vi "距离测量 - DS.vi"(7 "CSM Name":string="DS1") -> ()   [LabVIEW 2026, in "UI-距离测量.lvlib"]
uses:
  Supports/Sample Settings.ctl
  Data ColndSave/Supports/Time and Data.ctl
  TCP/Supports/UDP Settings.ctl
  <userlib>/_NEVSTOP/Communicable State Machine(CSM)/_Polymophic/CSM - Filter Duplicated Lines.vi
  aad2107a-5a5f-4fdf-8db0-9c36fd42b832.vi
  0bbdcba1-9d5b-49e3-b023-81a6ed1a833f.vi
  d3182339-f607-4847-9390-ad77bbb9bef6.vi
  a3283b4f-3d7d-475f-8286-b95f18be6a9d.vi
  b77c2947-8455-45d0-8563-f45fdc66c63a.vi
  c6692627-02fb-4556-9c5d-59e6097d0856.vi
  8c0fc226-3871-4866-9b38-f175316b3ef9.vi
  8417ea6c-3bd9-4cd5-8933-b29b0935beb3.vi
  <userlib>/_NEVSTOP/Communicable State Machine(CSM)/_Polymophic/CSM - Replace Marks in Messages.vi
  9e8a82e7-73dc-49c7-a8e1-da740b95007e.vi
  45363da5-0a68-41f0-863f-59b1647d93dc.vi
  684e6125-f2cc-419b-bab0-170e1ce567bd.vi
  5163a33a-69e0-492d-a74e-a390bdb1a610.vi
  3f58c0c9-4519-4815-81b6-823063e0ea10.vi
  ed6ed594-6bdd-4916-8b11-5c87dc2a661e.vi
  f090f7de-5b96-425f-bcc2-868efcdef004.vi
  7a757d38-3930-42d9-9f77-20f8f863129d.vi
  d1e74b47-9369-4dfd-ba75-b02d04b7ee9f.vi
  ba09a988-f7d6-44f3-a6d8-47fd2b4ee3b5.vi
  4c4982bb-7a2e-4137-8dbb-56eff7d2cb39.vi
  d32f4df3-bc1c-40d9-8b4f-fe0ac986a064.vi
  <userlib>/_NEVSTOP/Communicable State Machine(CSM)/AdvanceAPI/CSM - Compact Multiple States.vi
  <userlib>/_NEVSTOP/Communicable State Machine(CSM)/AdvanceAPI/CSM - Break Down Multiple States String.vi
  <userlib>/_NEVSTOP/Communicable State Machine(CSM)/_Shared/Remove Comments from Single-line.vi
  <userlib>/_NEVSTOP/Communicable State Machine(CSM)/_Shared/Split Single-line Message.vi
  <userlib>/_NEVSTOP/Communicable State Machine(CSM)/_Shared/Trim Single-line Text.vi
  <userlib>/_NEVSTOP/Communicable State Machine(CSM)/AdvanceAPI/CSM - Revert Arguments-Safe String.vi
  <userlib>/_NEVSTOP/Communicable State Machine(CSM)/AdvanceAPI/CSM - Make String Arguments Safe.vi
  c6692627-02fb-4556-9c5d-59e6097d0856.vi/99de0c97-112a-4c86-9094-c187659127e1.vi
  <userlib>/_NEVSTOP/Communicable State Machine(CSM)/Utility/Build Error Cluster.vi
  8417ea6c-3bd9-4cd5-8933-b29b0935beb3.vi/99de0c97-112a-4c86-9094-c187659127e1.vi
  <userlib>/_NEVSTOP/Communicable State Machine(CSM)/AdvanceAPI/CSM - Keywords.vi
  <userlib>/_NEVSTOP/Communicable State Machine(CSM)/addons/API-String-Arugments-Support/_Support/Data To API String Arguments.vi
  <userlib>/_NEVSTOP/Communicable State Machine(CSM)/addons/INI-Static-Variable-Support/_Support/instances/_CSM - Read File Logger Configuration - v1.0.vi
  <vilib>/Utility/Data Type/Get Type Information.vi
  <userlib>/_NEVSTOP/Communicable State Machine(CSM)/addons/API-String-Arugments-Support/_Support/Data To SingleElementsArray_csm.vi
  <userlib>/_NEVSTOP/Communicable State Machine(CSM)/addons/INI-Static-Variable-Support/_Support/Parse Used Session and Name.vi
  <userlib>/_NEVSTOP/Communicable State Machine(CSM)/addons/INI-Static-Variable-Support/_Support/INI-FGV(lvlibp).vi
  <userlib>/_NEVSTOP/Communicable State Machine(CSM)/addons/INI-Static-Variable-Support/_Support/Populate String with INI Variable.vi
  <userlib>/_NEVSTOP/Communicable State Machine(CSM)/addons/API-String-Arugments-Support/_Support/Convert API String Arguments to Data(variant).vi
  <userlib>/_NEVSTOP/Communicable State Machine(CSM)/addons/API-String-Arugments-Support/_Support/SingleElementsArray To Data_csm.vi
  <userlib>/_NEVSTOP/Communicable State Machine(CSM)/addons/MassData-Parameter/_support/FGV-MassData(lvlibp).vi
  <vilib>/Instr/_visa.llb/VISA Configure Serial Port (Instr).vi
  <userlib>/_NEVSTOP/Communicable State Machine(CSM)/Communicable State Machine.lvlib
  Acquisition/Acquisition.lvlib
  <userlib>/_NEVSTOP/Communicable State Machine(CSM)/addons/MassData-Parameter/CSM MassData Parameter Support.lvlib
  <userlib>/_NEVSTOP/Communicable State Machine(CSM)/addons/INI-Static-Variable-Support/INI-Static-Variable-Support.lvlib
  <userlib>/_NEVSTOP/Communicable State Machine(CSM)/addons/Watchdog/CSM Watchdog.lvlib
  <userlib>/_NEVSTOP/Communicable State Machine(CSM)/addons/Logger/CSM File Logger.lvlib
  Logging/Logging.lvlib
  Data ColndSave/Data Collection and Save.lvlib
  TCP/UDP.lvlib
panel:
  in  "停止":bool
  in  "温度显示":enum32{"距离测量", "Status"}(tab)
  in  "地址":string
  in  "UDP":bool
  in  "光功率模式":bool
  in  "光功率设置":u32
  in  "光开关":bool
  in  "距离采集开关":bool
  in  "USB Port":refnum<visa-resource-name>="COM3"
  in  "Interval(s)":dbl=0.5
  out "距离":waveform(dbl)(graph)
  in  "子程序？":bool
  out "Error Occurred":errorcluster caption="温度采集-错误输出"
  out "State History":string
  # "(5-1000)"
  # "mm"
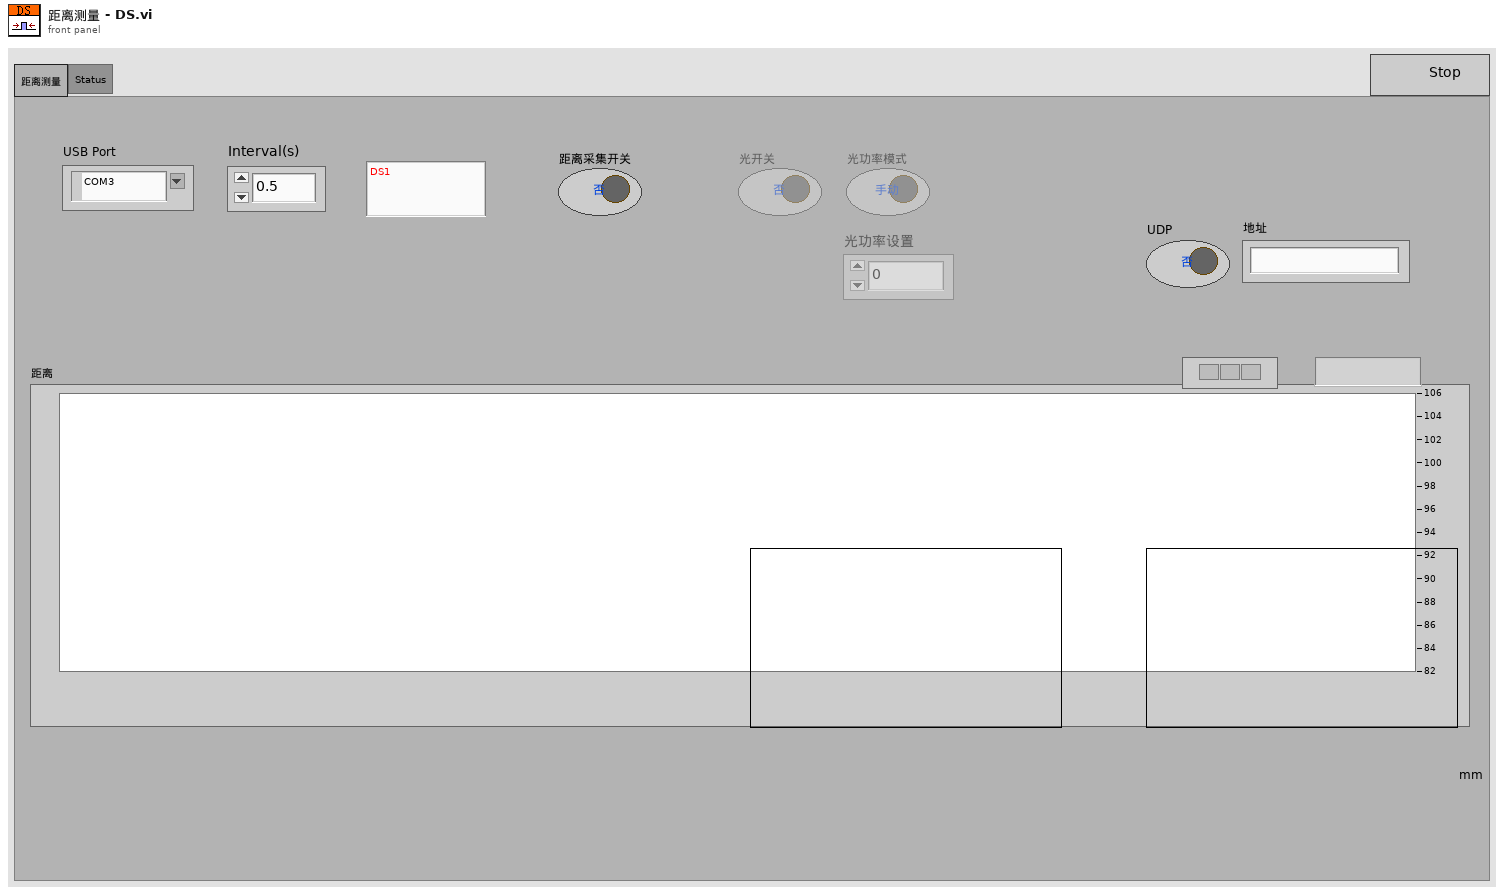
[diagram p1: front panel]
types:
  T1 = cluster{"Enable":bool, "Limit":cluster{"FileSize":i64, "FileNum":i32}, "Timestamp.Format":string, "AutoExit":bool}
  T2 = enum32{"Invalid", "Standard", "Closed", "Hidden", "Minimized", "Maximized"}
  T3 = enum32{"invalid app kind", "Development System", "Run Time System", "Student Edition", "Embedded LabVIEW", "Evaluation", "Custom"}
  T4 = cluster{"波特率":u32, "数据位":u16, "校验":enum16{"None", "Odd", "Even", "Mark", "Space"}, "停止位":u16, "流控制":u16}
  T5 = typedef "UI-距离测量.lvlib/读写指令类型.ctl" = enum16{"03读保持寄存器", "04读输入寄存器", "06写单个寄存器"}
  T6 = typedef "UI-距离测量.lvlib/UDP.lvlib/UDP Settings.ctl" = cluster{"连接ID":refnum<k16>, "网络地址(字符串)":string, "地址":u32, "本端口":u16, "对向":u16, "Read Interval":dbl, "Write Interval":dbl}
  T7 = typedef "Communicable State Machine.lvlib/_CSM_Response Source Message.ctl" = cluster{"‘State":string, "’Arguments":string, "’Error":errorcluster}
  T8 = cluster{"Current VI Reference":refnum<vi>, "Close Panel on Exit?":bool}
  T9 = typedef "UI-距离测量.lvlib/Sample Settings.ctl" = cluster{"USB Port":refnum<visa-resource-name>, "Interval(s)":dbl}
  T10 = typedef "Data Collection and Save.lvlib/Time and Data.ctl" = cluster{"采集时间":timestamp, "Data":dbl[]}
  T11 = cluster{"Core":cluster{"Current VI Reference":refnum<vi>, "Close Panel on Exit?":bool}, "Sample Settings":T9, "Time and Data":T10, "子程序？":bool}
  T12 = enum8{"Enabled", "Disabled", "Disabled and Grayed Out"}
  T13 = typedef "全局变量数据.ctl" = cluster{"温度采集":dbl[], "温度控制":dbl[], "压力测量":dbl[], "Zolix":dbl[], "步进电机":dbl[], "湿度测量":dbl[], "距离测量":dbl[]}
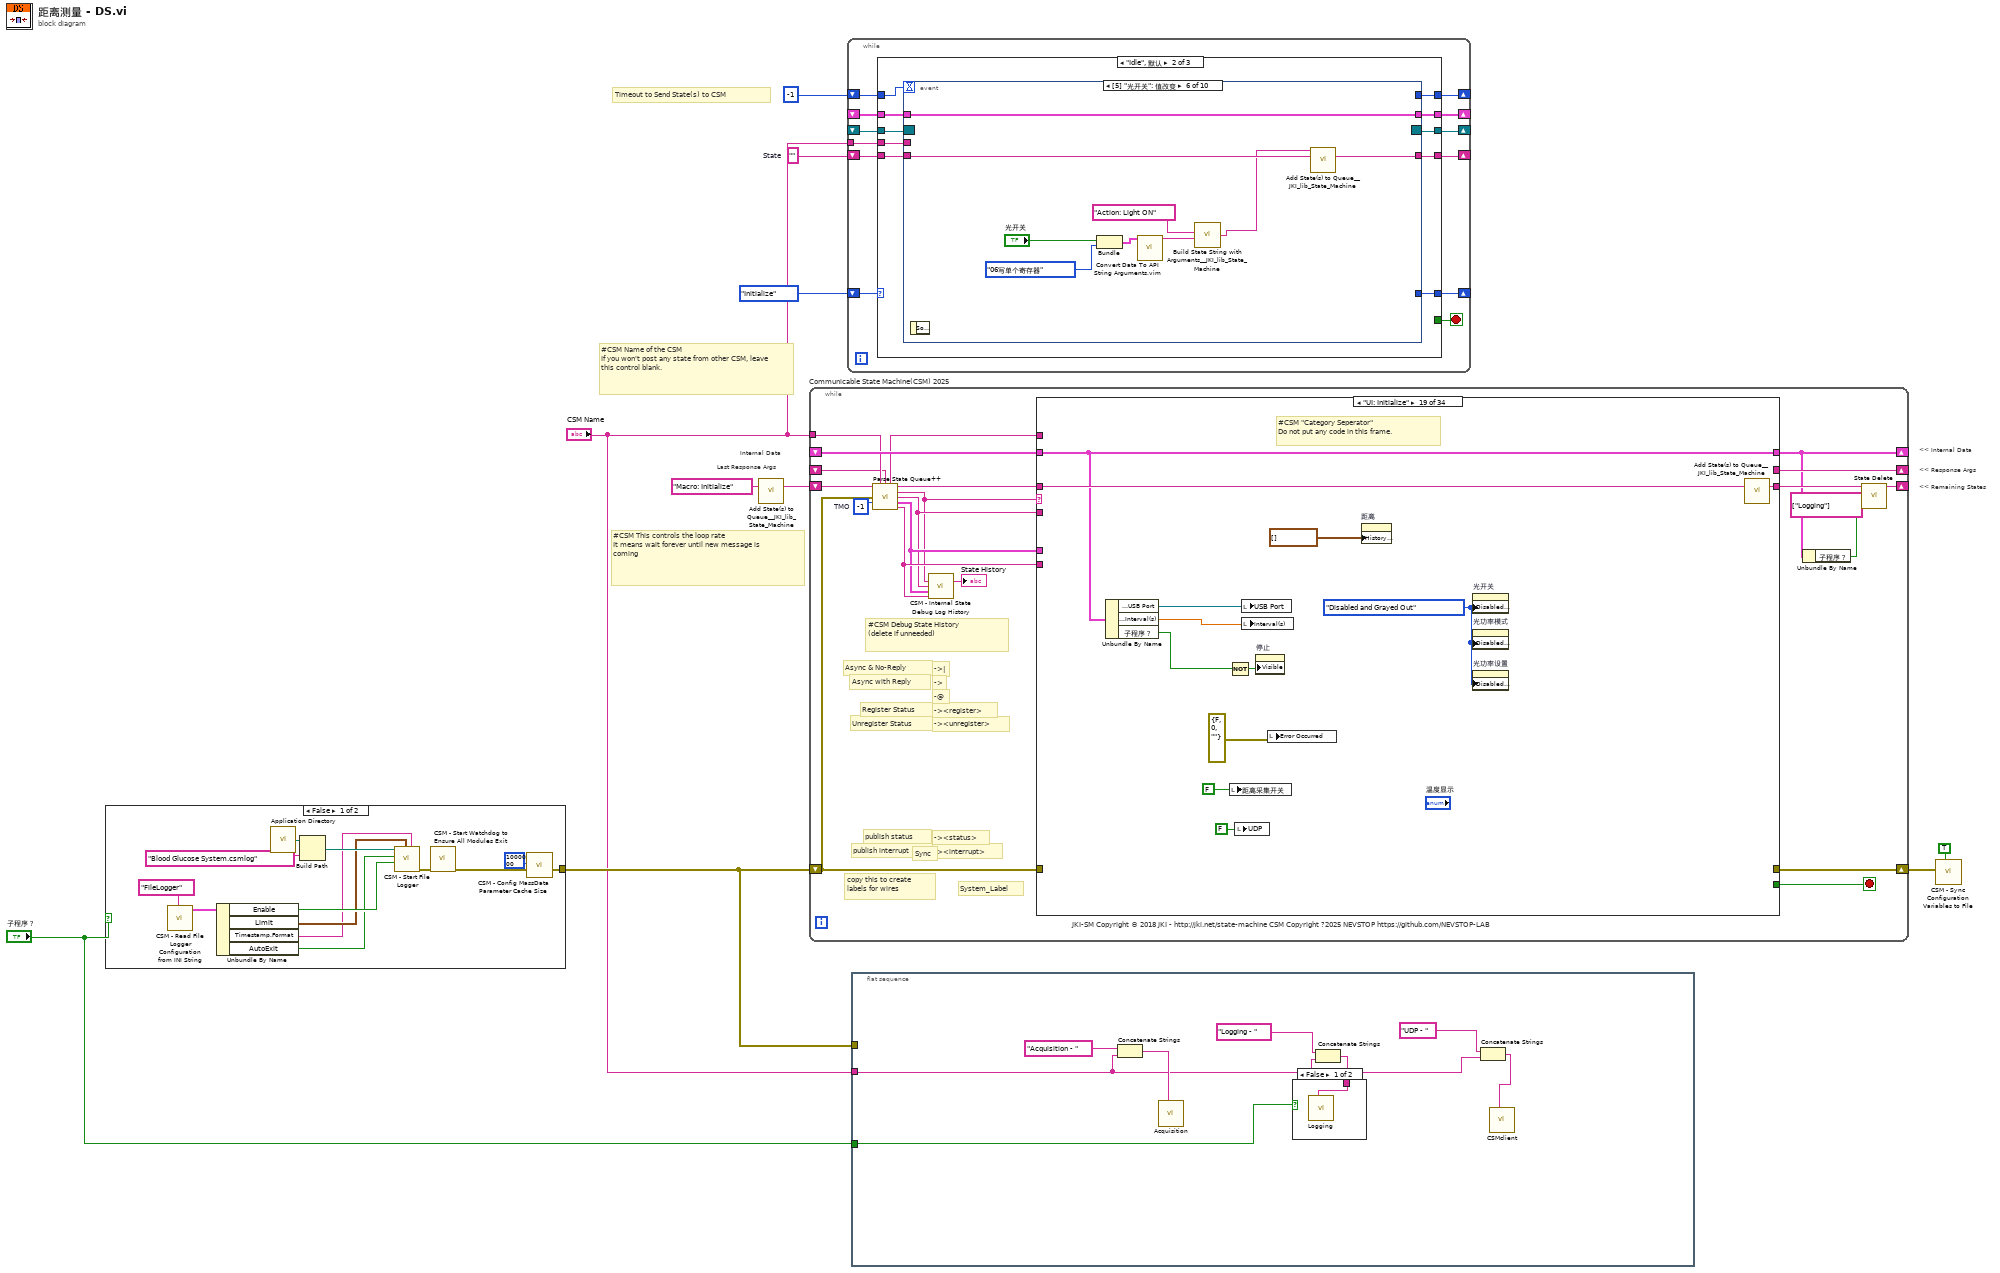
[diagram p0: block diagram]
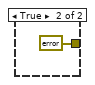
[diagram p2: hidden frame]
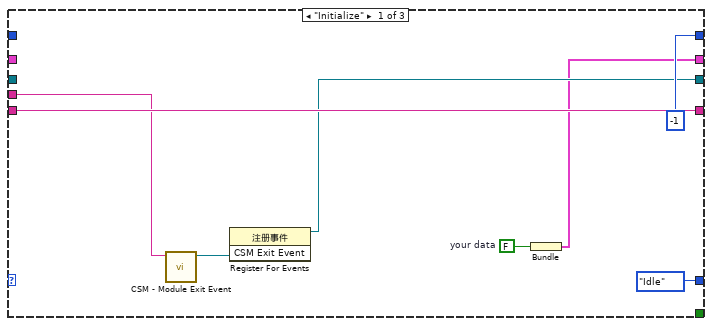
[diagram p4: hidden frame]
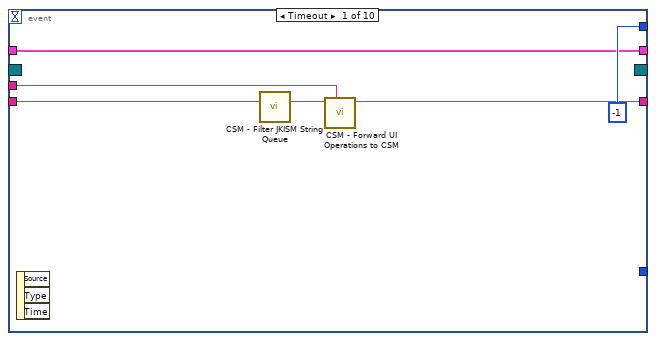
[diagram p5: hidden frame]
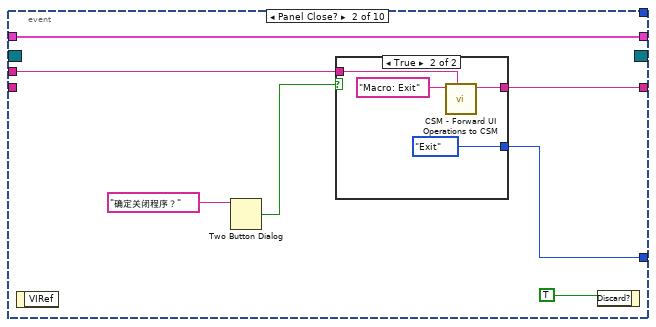
[diagram p6: hidden frame]
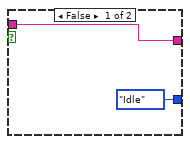
[diagram p7: hidden frame]
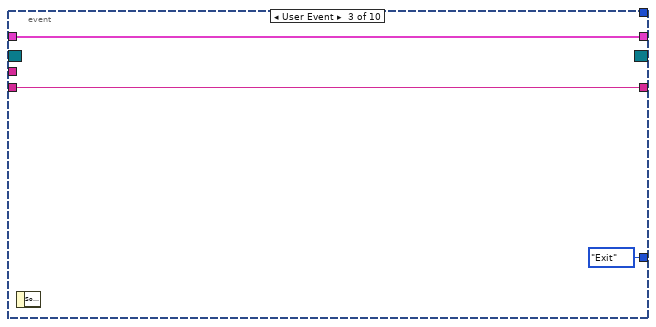
[diagram p8: hidden frame]
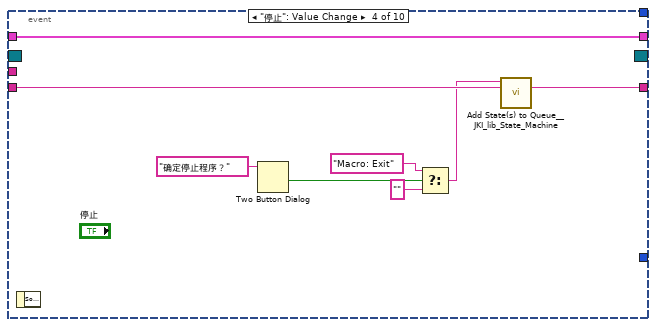
[diagram p9: hidden frame]
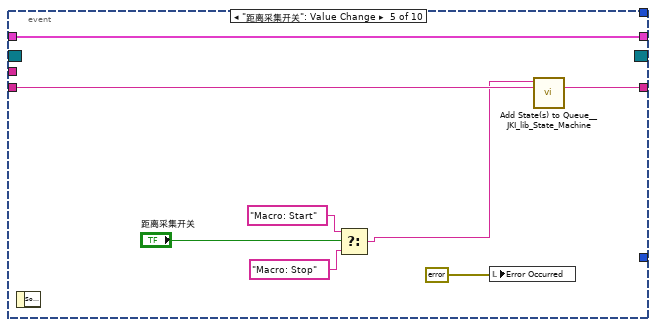
[diagram p10: hidden frame]
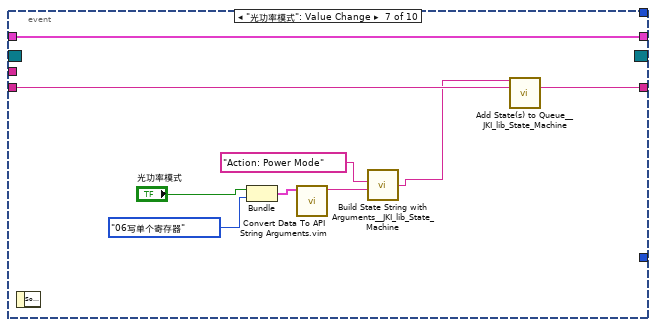
[diagram p11: hidden frame]
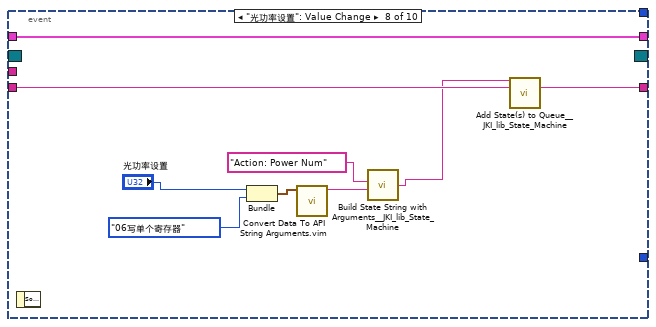
[diagram p12: hidden frame]
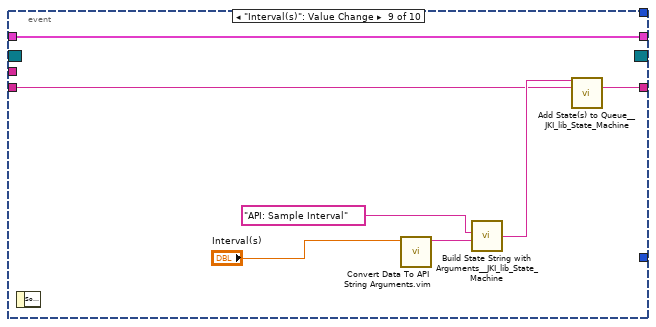
[diagram p13: hidden frame]
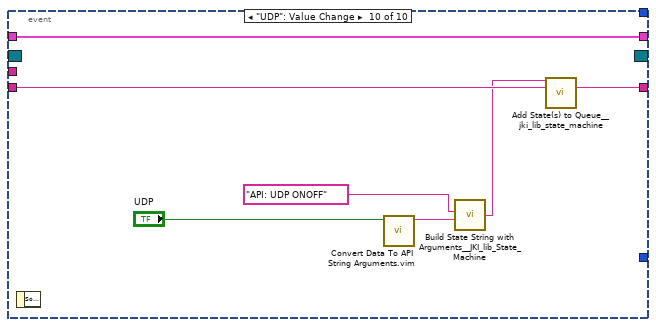
[diagram p14: hidden frame]
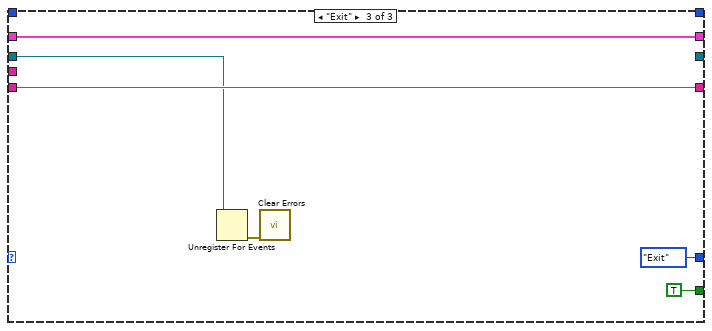
[diagram p15: hidden frame]
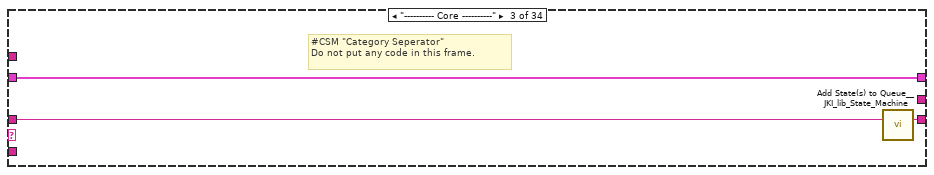
[diagram p18: hidden frame]
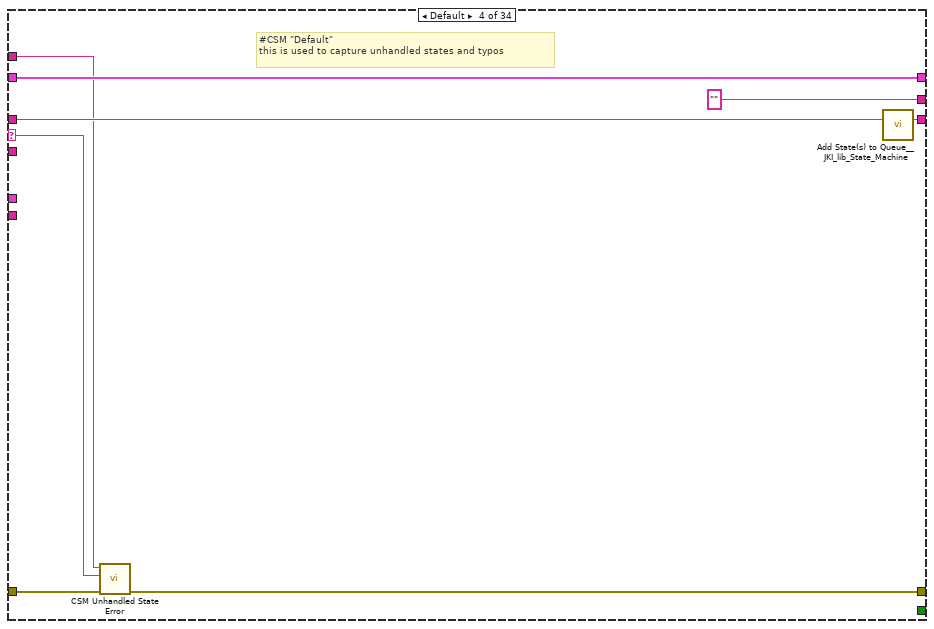
[diagram p19: hidden frame]
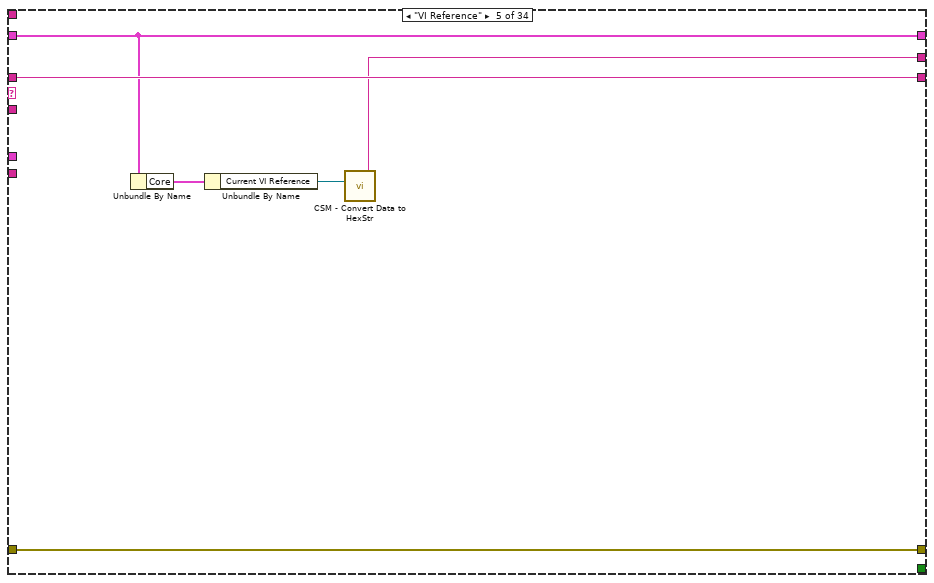
[diagram p20: hidden frame]
diagram:
  w9 = ""  # State
  # "Timeout to Send State(s) to CSM"
  # "Last Response Args"
  # "Internal Data"
  # "#CSM Name of the CSM\nIf you won't post any state from other CSM, leave this control blank."
  # "#CSM This controls the loop rate\nIt means wait forever until new message is coming"
  # "<< Internal Data"
  # "<< Response Args"
  # "<< Remaining States"
  n1 = case shown="False" "子程序？" {
    tunnel: [w11 errorcluster {"status"=FALSE, "code"=0, "source"=""} ("Error out")] -> w5
    frame False {
      n2 = call-poly <userlib>:"CSM - Read File Logger Configuration from INI String.vi"("Section Name(\"FileLogger\")"="FileLogger" ("Section Name(\"\" as Default)")) -> ("FileLogger Configuration-v1"=w18:T1)  [unwired: 7 in, 1 out]
      n3 = Unbundle By Name(w18) -> ("Enable"=w17:bool, "Limit"=w16:cluster{"FileSize":i64, "FileNum":i32}, "Timestamp.Format"=w14:string, "AutoExit"=w15:bool)
      n4 = call <vilib>:"Application Directory.vi"() -> ("Application Directory"=w23:path)
      n5 = Build Path(base path=w23, name or relative path="Blood Glucose System.csmlog") -> (appended path=w21:path)
      n6 = call <userlib>:"CSM - Start File Logger.vi"("Timestamp Format"=w14, "Log Limit"=w16, "Watchdog? (T)"=w17, "Exit When All Module Exist? (F)"=w15, "Log File Path"=w21) -> ("error out"=w20:errorcluster)  [unwired: 4 in, 2 out]
      n7 = call <userlib>:"CSM - Start Watchdog to Ensure All Modules Exit.vi"("error in (no error)"=w20) -> ("error out"=w12:errorcluster)  [unwired: 10 in]
      n8 = call <userlib>:"CSM - Config MassData Parameter Cache Size.vi"("Error in"=w12, "Size (50M)"=1000000 ("size(1M)")) -> ("Error out"=w11:errorcluster)  [unwired: 9 in]
    }
    frame True {
    }
  }
  n9 = call <vilib>:"Add State(s) to Queue__JKI_lib_State_Machine.vi"("State(s) in (\"\")"="Macro: Initialize" ("Init State(\"Macro: Initialize\")")) -> ("States Out"=w6:string)  [unwired: 14 in]
  n10 = while "Communicable State Machine(CSM) 2025" {
    shift-right: [w26] -> _
    shift-left: _ -> [w41]
    shift-right: [w43] -> w3
    shift-left: w5 -> [w31]
    shift-right: [w28] -> _
    shift-left: w6 -> [w44]
    tunnel: "CSM Name" -> [w38]
    shift-right: [w39] -> _
    shift-left: _ -> [w33]
    stop <- w42 stop-if-true
    w40 = -1  # TMO
    # "#CSM Debug State History\n(delete if unneeded)"
    # "-><interrupt>"
    # "-><status>"
    # "-><unregister>"
    # "-><register>"
    # "-@"
    # "->"
    # "->|"
    # "publish interrupt"
    # "publish status"
    # "Unregister Status"
    # "Register Status"
    # "Sync"
    # "Async with Reply"
    # "Async & No-Reply"
    # "JKI-SM Copyright © 2018 JKI - http://jki.net/state-machine CSM Copyright ?2025 NEVSTOP https://github.com/NEVSTOP-LAB"
    # "copy this to create labels for wires"
    # "System_Label"
    n11 = call <userlib>:"Parse State Queue++.vi"("State Queue"=w44, "Name (\"\" to Use UUID)"=w38, "Response Arguments"=w33, "Previous Error"=w31, "Dequeue (1 ms)"=w40) -> ("Name Used"=w32:string, "Remaining States"=w45:string, "Current State"=w34:string, "Arguments"=w35:string, "Additional Information"=w36:T7, "Source CSM"=w37:string)  [unwired: 5 in]
    n12 = call <userlib>:"CSM - Internal State Debug Log History.vi"("State"=w34, "Arguments (\"\")"=w35, ">> Response Source Message >>"=w36, "Source (\"\")"=w37) -> ("Debug Log"=→"State History":string)  [unwired: 11 in]
    n13 = case shown="\"UI: Initialize\"" w34 {
      selector: w34 -> [_ _ _ w56 _ _ _ _ _ _ _ _ _ _ _ _ _ _ _ _ _ _ _ _ _ _ _ _ _ _ _ _ _ _]
      tunnel: w45 -> [w46 w49 w52 w60 w65 w71 w96 w102 w108 w118 w125 w137 w141 w144 w155 w162 w173 w176 w188 w197 w200 w206 w222 w253 w260 w268 w270 w285 w300 w313 w315 w326 w341 w348]
      tunnel: w35 -> [_ _ _ _ _ w70 w92 w99 w105 w112 _ _ _ _ _ w160 _ _ _ _ _ _ _ _ _ _ _ w284 w299 w312 _ w321 w337 _]
      tunnel: w41 -> [w47 w48 w50 w58 w64 w76 w94 w100 w106 w116 w124 w131 w139 w142 _ w158 w168 w174 w177 w195 w198 w204 w238 w251 w257 w266 w269 w281 w297 w310 w317 w322 w338 w345]
      tunnel: [_ _ _ w53 w66 errorcluster {"status"=FALSE, "code"=0, "source"=""} ("error out") w89 w97 w103 w119 _ _ _ _ _ _ w169 _ _ _ _ _ w212 _ w256 _ _ w275 w291 w306 _ _ _ _] -> w43
      tunnel: w31 -> [_ _ _ w54 w66 w74 w90 w98 w104 _ _ _ _ _ _ _ w170 _ _ _ _ _ _ _ _ _ _ w276 w292 w307 _ _ _ _]
      tunnel: [w46 w49 w51 w59 w65 w72 w95 w101 w107 w117 w125 w136 w140 w143 w154 w161 w172 w175 w187 w196 w199 w205 w240 w252 w259 w267 w271 w286 w301 w314 w316 w327 w342 w349] -> w29
      tunnel: [_ _ _ _ _ _ TRUE _ _ _ _ _ TRUE _ _ _ _ _ _ _ _ _ _ _ _ _ _ _ _ _ _ _ _ _] -> w42
      tunnel: [w47 w48 w50 w58 w64 w76 w94 w100 w106 w115 w124 w135 w139 w142 w153 w157 w168 w174 w177 w195 w198 w204 w208 w251 w257 w266 w269 w281 w297 w310 w317 w318 w338 w345] -> w26
      tunnel: w37 -> [_ _ _ _ _ w69 _ _ _ w113 _ _ _ _ _ _ _ _ _ _ _ _ _ _ _ _ _ _ _ _ _ _ _ _]
      tunnel: w36 -> [_ _ _ _ _ w68 _ _ _ w114 _ _ _ _ _ _ _ _ _ _ _ _ _ _ _ _ _ _ _ _ _ _ _ _]
      tunnel: [_ _ _ "" w61 _ _ _ _ _ _ _ _ _ _ _ _ _ _ _ _ _ _ _ _ _ _ _ _ _ _ _ _ _] -> w39
      tunnel: w32 -> [_ _ _ w55 _ _ w91 _ _ _ _ _ _ _ w151 _ w165 _ _ _ _ w202 w235 w249 _ w264 _ _ _ _ _ w324 w340 w347]
      frame "", "Idle" {
        # "#CSM \"Idle/Event Handler\"\nexecutes when the state queue is empty"
      }
      frame "CSM Documentation" {
        # "#CSM State Syntax\n\n// Comment line, all text to the right of “//” will be ignored\n// Local Message Example\nDoSth: DoA >> Arguments\n\n// Sync Call Example\nAPI: xxxx >> Arguments -@ TargetModule\n\n// Async Call Example\nAPI: xxxx >> Arguments -> TargetModule\n\n// Async Call without Reply Example\nAPI: xxxx >> Arguments ->| TargetModule\n\n// Broadcast normal status:\nStatus >> StatusArguments  -><status>\n\n// Broadcast Interrupt status:\nInterrupt >> StatusArguments  -><interrupt>\n\n// Register Source Module's status to Handler Module\nStatus@Source Module >> Handler Module@Handler Module -><register>\n\n// Unegister Source Module's status\nStatus@Source Module >> Handler Module -><unregister>"
        # "#CSM README FIRST\n\nCommunicable State Machine(CSM) is a LabVIEW application framework that builds upon JKI State Machine(JKISM). It follows the pattern of JKISM and extends the keywords to describe message communication between modules, including concepts such as Sync-Message, Async-Message, Subscription/Unsubscription of status - essential elements for creating reusable code modules. For more information, please visit the CSM wiki: https://nevstop-lab.github.io/CSM-Wiki/\n\nFor instructions on JKI State Machine, visit: \n    http://jki.net/state-machine/\nFor information about CSM, visit: \n    https://github.com/NEVSTOP-LAB"
        # "#CSM \"Documentation\"\nCase for holding CSM Documenation"
      }
      frame "---------- Core ----------" {
        # "#CSM \"Category Seperator\"\nDo not put any code in this frame."
        n14 = call <vilib>:"Add State(s) to Queue__JKI_lib_State_Machine.vi"("State(s) in (\"\")"=w52) -> ("States Out"=w51:string)  [unwired: 14 in]
      }
      frame Default {
        # "#CSM \"Default\"\nthis is used to capture unhandled states and typos"
        n15 = call <userlib>:"CSM Unhandled State Error.vi"("error in (no error)"=w54, "Undefined State"=w56, "CSM Name"=w55) -> ("error out"=w53:errorcluster)  [unwired: 8 in]
        n16 = call <vilib>:"Add State(s) to Queue__JKI_lib_State_Machine.vi"("State(s) in (\"\")"=w60) -> ("States Out"=w59:string)  [unwired: 14 in]
      }
      frame "VI Reference" {
        n17 = Unbundle By Name(w64) -> ("Core"=w63:T8)
        n18 = Unbundle By Name(w63) -> ("Current VI Reference"=w62:refnum<vi>)
        n19 = call <userlib>:"CSM - Convert Data to HexStr.vi"("Variant"=w62) -> ("HEX String (0-9,A-F)"=w61:string)  [unwired: 8 in]
      }
      frame "Error Handler" {
        # "#CSM \"Error Handler\"\nYou can also output any states to clean-up after errors occur"
        # "Clear error"
        n20 = case shown="错误" w74 {
          selector: w74 -> [_ w83]
          tunnel: [w81 w85] -> w73
          tunnel: w71 -> [w81 w84]
          tunnel: w70 -> [w80 _]
          tunnel: w69 -> [_ _]
          tunnel: w68 -> [_ _]
          tunnel: [w78 w83] -> w67
          frame No Error {
            n21 = call <userlib>:"CSM - Convert Argument to Error.vi"("Argument"=w80) -> ("Error"=w79:errorcluster)  [unwired: 4 in]
            n22 = flat-sequence {
              tunnel: w79 -> [w82]
              tunnel: [w82] -> w78
              frame #0 {
              }
            }
          }
          frame Error {
            # "#CSM Internal Error Handler Case \nIf any error Occurred, \"Error Occurred\" \nstatus update will be broadcasted to system.\nParameter is Error Cluster."
            n23 = call <userlib>:"CSM - Convert Error to Argument.vi"("Error"=w83) -> ("Argument"=w87:string)  [unwired: 4 in]
            n24 = call <vilib>:"Build State String with Arguments__JKI_lib_State_Machine.vi"("Arguments (\"\")"=w87, "State"="Error Occurred" ("Status with Arguments")) -> ("State with Arguments"=w86:string)  [unwired: 4 in]
            n25 = call <userlib>:"CSM - Broadcast Status Change.vi"("Status With Arguments"=w86, "State Queue"=w84) -> ("Remaining States"=w85:string)  [unwired: 13 in]
          }
        }
        "Error Occurred" <- w67
        n26 = call <vilib>:"Add State(s) to Queue__JKI_lib_State_Machine.vi"("State(s) in Front (\"\")"="// Post Error States", "State(s) in (\"\")"=w73) -> ("States Out"=w72:string)  [unwired: 13 in]
      }
      frame "Critical Error" {
        # "#CSM \"Critical Error\"\nWhen any un-recoverable error occurs, CSM goes into this case."
        # "#CSM Stop in Critical Error\nWhen Critical Error occurs, Stop the loop immediately. Do NOT change this unless you fully understand the impact."
        n27 = call <userlib>:"CSM Critical Error.vi"("error in (no error)"=w90, "Arugments (As Reason)"=w92, "CSM Name"=w91) -> ("error out"=w89:errorcluster)  [unwired: 8 in]
        n28 = call <vilib>:"Add State(s) to Queue__JKI_lib_State_Machine.vi"("State(s) in (\"\")"=w96) -> ("States Out"=w95:string)  [unwired: 14 in]
      }
      frame "Target Timeout Error" {
        # "#CSM \"Target Timeout Error\"\nWhen This CSM could not get the sync-call response in time, This CSM goes into this case."
        n29 = call <userlib>:"CSM Target Timeout Error.vi"("error in (no error)"=w98, "Arguments (As CSM Name)"=w99) -> ("error out"=w97:errorcluster)  [unwired: 9 in]
        n30 = call <vilib>:"Add State(s) to Queue__JKI_lib_State_Machine.vi"("State(s) in (\"\")"=w102) -> ("States Out"=w101:string)  [unwired: 14 in]
      }
      frame "Target Error" {
        # "#CSM \"Target Error\"\nWhen This CSM try to communicate with an un-existed CSM, This CSM goes into this case."
        n31 = call <userlib>:"CSM Target Error.vi"("error in (no error)"=w104, "Arguments (As CSM Name)"=w105) -> ("error out"=w103:errorcluster)  [unwired: 9 in]
        n32 = call <vilib>:"Add State(s) to Queue__JKI_lib_State_Machine.vi"("State(s) in (\"\")"=w108) -> ("States Out"=w107:string)  [unwired: 14 in]
      }
      frame "Async Response", "Response" {
        n33 = Unbundle(w114) -> ("‘State"=w111:string, "’Arguments"=w110:string, "’Error"=w109:errorcluster)
        n34 = case shown="默认" w111 {
          tunnel: [w120] -> w117
          tunnel: w118 -> [w121]
          tunnel: [w123] -> w115
          tunnel: w116 -> [w123]
          tunnel: [w122] -> w119
          tunnel: w109 -> [w122]
          tunnel: w113 -> [_]
          tunnel: w112 -> [_]
          tunnel: w110 -> [_]
          frame 默认 {
            # "#CSM \"Async Response\"\nHandle Async-call Response (\"Async Response\" for ->)"
            # "#CSM \"Response\"\nHandle Sync-call Response (\"Response\" for -@)"
            # "#CSM Response Comments\nAfter Message is executed, CSM goes to this state for receive the response.\n    For Async Message(->), \"Async Response\" is used. This CSM will goes to \"Async Message Posted\" immediately and receive the \"Async Response\" after the callee finishes the message.\n    For Sync Message(@),  This CSM will wait until the message is done and immediately goes to \"Response\""
            n35 = call <vilib>:"Add State(s) to Queue__JKI_lib_State_Machine.vi"("State(s) in (\"\")"=w121) -> ("States Out"=w120:string)  [unwired: 14 in]
          }
        }
      }
      frame "Async Message Posted" {
        # "#CSM \"Async Message Posted\"\nAfter Async Message is posted (-> or ->| ), CSM goes to this state for post-action.\nYou can use Argument - State to tell which Async Message is called."
      }
      frame "Initialize Core Data" {
        # "#CSM \"Initialize Core Data\"\nThis is used to determine panel behavior on exit"
        # "originally closed?"
        # "exe?"
        # "If panel starts closed or is an EXE, then close it when we exit"
        n36 = property class="VI"() -> ("FP.State"=w128:T2)  [unwired: 2 in, 2 out]
        n37 = property class="App"() -> ("App.Kind"=w134:T3)  [unwired: 2 in, 2 out]
        n38 = control-ref of="Current VI Reference"() -> (w129:refnum<vi>)
        n39 = Equal?(x=w128, y=T2."Closed" ("Front Panel Window:State")) -> (x = y?=w126:bool)
        n40 = Equal?(x=w134, y=T3."Run Time System" ("Application:Kind")) -> (x = y?=w132:bool)
        n41 = Or(x=w126, y=w132) -> (x .or. y?=w130:bool)
        n42 = Bundle By Name(cluster=w131, "Core.Current VI Reference"=w129, "Core.Close Panel on Exit?"=w130) -> (w135:T11)
        n43 = call <vilib>:"Add State(s) to Queue__JKI_lib_State_Machine.vi"("State(s) in (\"\")"=w137) -> ("States Out"=w136:string)  [unwired: 14 in]
      }
      frame "Exit" {
        # "#CSM \"Exit\"\nCase for exiting the loop. No errors that occur here will be handled."
        n44 = call <vilib>:"Add State(s) to Queue__JKI_lib_State_Machine.vi"("State(s) in (\"\")"=w141) -> ("States Out"=w140:string)  [unwired: 14 in]
      }
      frame "---------- Data ----------" {
        # "#CSM \"Category Seperator\"\nDo not put any code in this frame."
        n45 = call <vilib>:"Add State(s) to Queue__JKI_lib_State_Machine.vi"("State(s) in (\"\")"=w144) -> ("States Out"=w143:string)  [unwired: 14 in]
      }
      frame "Data: Initialize" {
        w145 = T10 {"采集时间"=timestamp(0 s since 1904-01-01), "Data"=[0.0]}  # Time and Data
        w147 = T9 {"USB Port"="COM3", "Interval(s)"=0.5}  # Sample Settings
        w152 = T8 {"Current VI Reference"=refnum, "Close Panel on Exit?"=FALSE}  # Core
        # "#CSM \"Data: Initialize\"\nInitialize the shift-register data, here.\n(data names are defined by what you wire into the bundle function)"
        # "#CSM do not delete - used by framework"
        # "#CSM Add new data here."
        # "#CSM Data names and types of shift register data are defined by this bundle."
        n46 = local read "子程序？"() -> (w150:bool)
        n47 = call "CSM - Read Cluster Elements From Session.vim"("Section Name (\"\" as Default)"=w151, "Cluster"=w147) -> ("Cluster out"=w148:T9)  [unwired: 6 in, 1 out]
        n48 = Select(t=w148, s=TRUE, f=w147) -> (s? t:f=w146:T9)
        n49 = Bundle("Core"=w152, "Sample Settings"=w146, "Time and Data"=w145, "子程序？"=w150) -> (w153:T11)  [unwired: 1 in]
        n50 = call <vilib>:"Add State(s) to Queue__JKI_lib_State_Machine.vi"("State(s) in (\"\")"=w155) -> ("States Out"=w154:string)  [unwired: 14 in]
      }
      frame "Data: Update Indicators" {
        w159 = T10 {"采集时间"=timestamp(0 s since 1904-01-01), "Data"=[]}  # Time and Data
        n51 = call "CSM - Convert Argument to MassData.vim"("Type"=w159, "MassData Argument"=w160) -> ("Data"=w156:T10)  [unwired: 6 in, 1 out]
        n52 = in-place {
          in-place-border: w156 -> [w164]
          n53 = in-place-cluster #1(w158) -> ()  [unwired: 1 out]
          n54 = in-place-cluster #1("Time and Data"=w164) -> (w157:T11)
        }
        n55 = call <vilib>:"Add State(s) to Queue__JKI_lib_State_Machine.vi"("State(s) in Front (\"\")"="UI: Update Graph" ("State(s) in Front (\"\")"), "State(s) in (\"\")"=w162) -> ("States Out"=w161:string)  [unwired: 13 in]
      }
      frame "Data: Cleanup" {
        # "#CSM \"Data: Cleanup\"\nCleanup any data and references, here.\n(this is called automatically, by the Macro: Exit)"
        n56 = Unbundle By Name(w168) -> ("Core.Current VI Reference"=w171:refnum<vi>, "Sample Settings"=w166:T9)
        n57 = call "CSM - Write Configuration Variable.vim"("Section Name (\"\" as Default)"=w165, "Configuration"=w166) -> ()  [unwired: 6 in, 2 out]
        n58 = Close Reference(reference=w171, error in (no error)=w170) -> (error out=w169:errorcluster)
        n59 = local write "距离采集开关"(FALSE ("温度采集开关")) -> ()
        n60 = call <vilib>:"Add State(s) to Queue__JKI_lib_State_Machine.vi"("State(s) in (\"\")"=w173) -> ("States Out"=w172:string)  [unwired: 14 in]
      }
      frame "---------- UI ----------" {
        # "#CSM \"Category Seperator\"\nDo not put any code in this frame."
        n61 = call <vilib>:"Add State(s) to Queue__JKI_lib_State_Machine.vi"("State(s) in (\"\")"=w176) -> ("States Out"=w175:string)  [unwired: 14 in]
      }
      frame "UI: Initialize" {
        w178 = T12."Disabled and Grayed Out" ("禁用")
        # "#CSM \"Category Seperator\"\nDo not put any code in this frame."
        n62 = Unbundle By Name(w177) -> ("Sample Settings.USB Port"=w184:refnum<visa-resource-name>, "Sample Settings.Interval(s)"=w183:dbl, "子程序？"=w182:bool)
        n63 = Not(x=w182) -> (.not. x?=w185:bool)
        n64 = local write "距离采集开关"(FALSE ("温度采集开关")) -> ()
        n65 = local write "UDP"(FALSE ("UDP")) -> ()
        n66 = local write "USB Port"(w184) -> ()
        n67 = local write "Interval(s)"(w183) -> ()
        n68 = property on="停止" class="Bool"("Visible"=w185) -> ()  [unwired: 2 in, 2 out]
        n69 = local write "Error Occurred"(errorcluster {"status"=FALSE, "code"=0, "source"=""} ("Error Occurred")) -> ()
        n70 = property on="距离" class="WFChart (严格)"("History Data"=waveform(dbl)[] [] ("历史数据")) -> ()  [unwired: 2 in, 2 out]
        n71 = property on="光开关" class="Bool (严格)"("DisabledEnum"=w178) -> ()  [unwired: 2 in, 2 out]
        n72 = property on="光功率模式" class="Bool (严格)"("DisabledEnum"=w178) -> ()  [unwired: 2 in, 2 out]
        n73 = property on="光功率设置" class="DigNum (严格)"("DisabledEnum"=w178) -> ()  [unwired: 2 in, 2 out]
        n74 = call <vilib>:"Add State(s) to Queue__JKI_lib_State_Machine.vi"("State(s) in (\"\")"=w188) -> ("States Out"=w187:string)  [unwired: 14 in]
      }
      frame "UI: Update Graph" {
        # "#CSM \"Category Seperator\"\nDo not put any code in this frame."
        n75 = Unbundle By Name(w195) -> ("Time and Data.Data"=w189:dbl[], "Time and Data.采集时间"=w194:timestamp, "Sample Settings.Interval(s)"=w193:dbl)
        n76 = global read "辅助系统全局变量 - T1.vi" "温度相关数据"() -> (w190:T13)
        n77 = Bundle By Name(cluster=w190, "距离测量"=w189) -> (w191:T13)
        n78 = Bundle By Name("Y"=w189, "t0"=w194, "dt"=w193) -> (→"距离":waveform(dbl))  [unwired: 1 in]
        n79 = global write "辅助系统全局变量 - T1.vi" "温度相关数据"(w191) -> ()
        n80 = call <vilib>:"Add State(s) to Queue__JKI_lib_State_Machine.vi"("State(s) in (\"\")"=w197) -> ("States Out"=w196:string)  [unwired: 14 in]
      }
      frame "---------- Macro ----------" {
        # "#CSM \"Category Seperator\"\nDo not put any code in this frame."
        n81 = call <vilib>:"Add State(s) to Queue__JKI_lib_State_Machine.vi"("State(s) in (\"\")"=w200) -> ("States Out"=w199:string)  [unwired: 14 in]
      }
      frame "Macro: Initialize" {
        w203 = "Data: Initialize\nInitialize Core Data\nUI: Initialize\n\n//Permanent registrations\nAcquired Data@Acquisition - <1> >> Data: Update Indicators -><register>\nAcquired Data@Acquisition - <1> >> API: Log@Logging - <1> -><register>\n\n//Error registrations\nError Occurred@Acquisition - <1> >> Error Handler -><register>\nError Occurred@Logging - <1> >> Error Handler -><register>\n\n//Launch Acquisition Module\n"  # Data: Initialize Initialize Core Data UI: Initialize  //Permanent registrations Acquired Data@Acquisition - <1> >> Data: Update Indicators -><register> Acquired Data@Acquisition - <1> >> API: Log@Logging - <1> -><register>  //Error registrations Error Occurred@Acquisition - <1> >> Error Handler -><register> Error Occurred@Logging - <1> >> Error Handler -><register>  //Launch Acquisition Module
        # "#CSM \"Macro: Initialize\"\nInitialization Macro (This is called once, when the VI starts)"
        n82 = call-poly <userlib>:"Build Message with Arguments++.vi"("States With Replace Token"=w203, "<1>"=w202) -> ("States"=w201:string)  [unwired: 13 in]
        n83 = call <vilib>:"Add State(s) to Queue__JKI_lib_State_Machine.vi"("State(s) in Front (\"\")"=w201, "State(s) in (\"\")"=w206) -> ("States Out"=w205:string)  [unwired: 13 in]
      }
      frame "Macro: Start" {
        w209 = T12."Enabled" ("禁用")
        n84 = local write "距离采集开关"(TRUE ("温度采集开关")) -> ()
        n85 = Unbundle By Name(T4 {"波特率"=115200, "数据位"=8, "校验"=enum."None", "停止位"=10, "流控制"=0} ("串口设置")) -> ("波特率"=w216:u32, "数据位"=w217:u16, "校验"=w218:enum16{"None", "Odd", "Even", "Mark", "Space"}, "停止位"=w219:u16, "流控制"=w220:u16)
        n86 = call-poly "VISA Configure Serial Port"("VISA resource name"="USB Port", "timeout (10sec)"=u32 3000, "baud rate (9600)"=w216, "data bits (8)"=w217, "parity (0:none)"=w218, "stop bits (10: 1 bit)"=w219, "flow control (0:none)"=w220) -> ("VISA resource name out"=w207:refnum<visa-resource-name>, "error out"=w212:errorcluster)  [unwired: 2 in, 5 out]
        n87 = Bundle By Name(cluster=w238, "Sample Settings.USB Port"=w207) -> (w208:T11)
        n88 = Unbundle By Name(w208) -> ("Sample Settings"=w239:T9)
        n89 = call "Convert Data To API String Arguments.vim"("Data"=cluster{"光功率模式":bool, "写/读":T5} {"光功率模式"=FALSE, "写/读"=enum."03读保持寄存器"} ("簇")) -> ("API String"=w231:string)  [unwired: 7 in, 1 out]
        n90 = call "Convert Data To API String Arguments.vim"("Data"=cluster{"光开关":bool, "写/读":T5} {"光开关"=TRUE, "写/读"=enum."06写单个寄存器"} ("簇")) -> ("API String"=w233:string)  [unwired: 7 in, 1 out]
        n91 = call "Convert Data To API String Arguments.vim"("Data"=cluster{"光功率设置":u32, "写/读":T5} {"光功率设置"=0, "写/读"=enum."03读保持寄存器"} ("簇")) -> ("API String"=w232:string)  [unwired: 7 in, 1 out]
        n92 = call "Convert Data To API String Arguments.vim"("Data"=w239) -> ("API String"=w236:string)  [unwired: 7 in, 1 out]
        n93 = call <vilib>:"Build State String with Arguments__JKI_lib_State_Machine.vi"("Arguments (\"\")"=w232, "State"="Action: Power Num") -> ("State with Arguments"=w223:string)  [unwired: 4 in]
        n94 = call <vilib>:"Build State String with Arguments__JKI_lib_State_Machine.vi"("Arguments (\"\")"=w231, "State"="Action: Power Mode") -> ("State with Arguments"=w224:string)  [unwired: 4 in]
        n95 = call <vilib>:"Build State String with Arguments__JKI_lib_State_Machine.vi"("Arguments (\"\")"=w233, "State"="Action: Light ON") -> ("State with Arguments"=w210:string)  [unwired: 4 in]
        n96 = call-poly <userlib>:"Build Message with Arguments++.vi"("States With Replace Token"="API: Start >> <param> -@ Acquisition - <1>\nAPI: Start  -@ Logging - <1>" ("State"), "<param>"=w236, "<1>"=w235) -> ("States"=w211:string)  [unwired: 12 in]
        n97 = call <vilib>:"Add State(s) to Queue__JKI_lib_State_Machine.vi"("State(s) in Front (\"\")"=w211, "State(s) in (\"\")"=w224, "State(s) at Back (\"\")"=w223) -> ("States Out"=w221:string)  [unwired: 12 in]
        n98 = property on="光开关" class="Bool (严格)"("DisabledEnum"=w209) -> ()  [unwired: 2 in, 2 out]
        n99 = property on="光功率模式" class="Bool (严格)"("DisabledEnum"=w209) -> ()  [unwired: 2 in, 2 out]
        n100 = property on="光功率设置" class="DigNum (严格)"("DisabledEnum"=w209) -> ()  [unwired: 2 in, 2 out]
        n101 = call <vilib>:"Add State(s) to Queue__JKI_lib_State_Machine.vi"("State(s) in Front (\"\")"=w210, "State(s) in (\"\")"=w221, "State(s) at Back (\"\")"=w222) -> ("States Out"=w240:string)  [unwired: 12 in]
      }
      frame "Macro: Stop" {
        # "#CSM \"Macro: Exit\"\nExit Macro (This is called once, when the VI exits)"
        n102 = local write "距离采集开关"(FALSE ("温度采集开关")) -> ()
        n103 = call "Convert Data To API String Arguments.vim"("Data"=cluster{"光开关":bool, "写/读":T5} {"光开关"=FALSE, "写/读"=enum."06写单个寄存器"} ("簇")) -> ("API String"=w247:string)  [unwired: 7 in, 1 out]
        n104 = call <vilib>:"Build State String with Arguments__JKI_lib_State_Machine.vi"("Arguments (\"\")"=w247, "State"="Action: Light ON") -> ("State with Arguments"=w242:string)  [unwired: 4 in]
        n105 = call-poly <userlib>:"Build Message with Arguments++.vi"("States With Replace Token"="//Send Message to Other CSM Modules\nAPI: Stop -@ Acquisition - <1>\nAPI: Stop -@ Logging - <1>\n", "<1>"=w249) -> ("States"=w243:string)  [unwired: 13 in]
        n106 = call <vilib>:"Add State(s) to Queue__jki_lib_state_machine.vi"("State(s) in Front (\"\")"=w243, "State(s) in (\"\")"=w242, "State(s) at Back (\"\")"="Macro: Close") -> ("States Out"=w244:string)  [unwired: 12 in]
        n107 = call <vilib>:"Add State(s) to Queue__JKI_lib_State_Machine.vi"("State(s) in Front (\"\")"=w244, "State(s) in (\"\")"=w253) -> ("States Out"=w252:string)  [unwired: 13 in]
      }
      frame "Macro: Close" {
        # "#CSM \"Macro: Exit\"\nExit Macro (This is called once, when the VI exits)"
        n108 = Unbundle By Name(w257) -> ("Sample Settings.USB Port"=w258:refnum<visa-resource-name>)
        n109 = call "Stall Data Flow.vim"("value in"=w258, "milliseconds to wait"=u32 150) -> ("value out"=w255:refnum<visa-resource-name>)  [unwired: 1 out]
        n110 = VISA Close(VISA resource name=w255) -> (error out=w256:errorcluster)  [unwired: 1 in]
        n111 = call <vilib>:"Add State(s) to Queue__JKI_lib_State_Machine.vi"("State(s) in (\"\")"=w260) -> ("States Out"=w259:string)  [unwired: 14 in]
      }
      frame "Macro: Exit" {
        w265 = "//Exit\nMacro: Exit-@Acquisition - <1>\nMacro: Exit-@Logging - <1>\nAPI: UDP Exit\n\n//Permanent unregistrations\nAcquired Data@Acquisition - <1> >> Data: Update Indicators -><unregister>\nAcquired Data@Acquisition - <1> >> API: Log@Logging - <1> -><unregister>\n\n//Permanent unregistrations\nError Occurred@Acquisition - <1> >> Error Handler -><unregister>\nError Occurred@Logging - <1> >> Error Handler -><unregister>\n"  # //Exit Macro: Exit-@Acquisition - <1> Macro: Exit-@Logging - <1> API: UDP Exit  //Permanent unregistrations Acquired Data@Acquisition - <1> >> Data: Update Indicators -><unregister> Acquired Data@Acquisition - <1> >> API: Log@Logging - <1> -><unregister>  //Permanent unregistrations Error Occurred@Acquisition - <1> >> Error Handler -><unregister> Error Occurred@Logging - <1> >> Error Handler -><unregister>
        # "#CSM \"Macro: Exit\"\nExit Macro (This is called once, when the VI exits)"
        n112 = call-poly <userlib>:"Build Message with Arguments++.vi"("States With Replace Token"=w265, "<1>"=w264) -> ("States"=w262:string)  [unwired: 13 in]
        n113 = call <vilib>:"Add State(s) to Queue__JKI_lib_State_Machine.vi"("State(s) in Front (\"\")"=w262, "State(s) at Back (\"\")"="Macro: Close\nData: Cleanup\nExit") -> ("States Out"=w263:string)  [unwired: 13 in]
        n114 = call <vilib>:"Add State(s) to Queue__JKI_lib_State_Machine.vi"("State(s) in Front (\"\")"=w263, "State(s) in (\"\")"=w268) -> ("States Out"=w267:string)  [unwired: 13 in]
      }
      frame "---------- Action ----------" {
        # "#CSM \"Category Seperator\"\nDo not put any code in this frame."
        n115 = call <vilib>:"Add State(s) to Queue__JKI_lib_State_Machine.vi"("State(s) in (\"\")"=w270) -> ("States Out"=w271:string)  [unwired: 14 in]
      }
      frame "Action: Light ON" {
        # "#CSM \"Category Seperator\"\nDo not put any code in this frame."
        n116 = call "Convert API String Arguments to Data.vim"("Reference Type"=cluster{"光开关":bool, "写/读":T5} {"光开关"=FALSE, "写/读"=enum."03读保持寄存器"} ("簇"), "API String"=w284) -> ("Data"=w282:cluster{"光开关":bool, "写/读":T5})  [unwired: 6 in, 1 out]
        n117 = Unbundle By Name(w281) -> ("Sample Settings.USB Port"=w280:refnum<visa-resource-name>)
        n118 = Unbundle By Name(w282) -> ("写/读"=w277:T5, "光开关"=w279:bool)
        n119 = Boolean To (0,1)(Boolean=w279) -> (0, 1=w278:i16)
        n120 = call "串口读写 - DS.vi"("寄存器地址"=u8 0, "错误输入（无错误）"=w276, "写入数据"=w278, "写/读"=w277, "VISA输入"=w280) -> ("错误输出"=w275:errorcluster, "读取设备(n)"=w273:i32)  [unwired: 4 in, 1 out]
        n121 = Greater Than 0?(x=w273) -> (x > 0?=w274:bool)
        n122 = local write "光开关"(w274) -> ()
        n123 = call <vilib>:"Add State(s) to Queue__JKI_lib_State_Machine.vi"("State(s) in (\"\")"=w285) -> ("States Out"=w286:string)  [unwired: 14 in]
      }
      frame "Action: Power Mode" {
        # "#CSM \"Category Seperator\"\nDo not put any code in this frame."
        n124 = call "Convert API String Arguments to Data.vim"("Reference Type"=cluster{"光功率模式":bool, "写/读":T5} {"光功率模式"=FALSE, "写/读"=enum."03读保持寄存器"} ("簇"), "API String"=w299) -> ("Data"=w298:cluster{"光功率模式":bool, "写/读":T5})  [unwired: 6 in, 1 out]
        n125 = Unbundle By Name(w297) -> ("Sample Settings.USB Port"=w296:refnum<visa-resource-name>)
        n126 = Unbundle By Name(w298) -> ("写/读"=w293:T5, "光功率模式"=w295:bool)
        n127 = Boolean To (0,1)(Boolean=w295) -> (0, 1=w294:i16)
        n128 = call "串口读写 - DS.vi"("寄存器地址"=u8 1, "错误输入（无错误）"=w292, "写入数据"=w294, "写/读"=w293, "VISA输入"=w296) -> ("错误输出"=w291:errorcluster, "读取设备(n)"=w290:i32)  [unwired: 4 in, 1 out]
        n129 = Greater Than 0?(x=w290) -> (x > 0?=w287:bool)
        n130 = local write "光功率模式"(w287) -> ()
        n131 = call <vilib>:"Add State(s) to Queue__JKI_lib_State_Machine.vi"("State(s) in (\"\")"=w300) -> ("States Out"=w301:string)  [unwired: 14 in]
      }
      frame "Action: Power Num" {
        # "#CSM \"Category Seperator\"\nDo not put any code in this frame."
        n132 = call "Convert API String Arguments to Data.vim"("Reference Type"=cluster{"光功率设置":u32, "写/读":T5} {"光功率设置"=0, "写/读"=enum."03读保持寄存器"} ("簇"), "API String"=w312) -> ("Data"=w311:cluster{"光功率设置":u32, "写/读":T5})  [unwired: 6 in, 1 out]
        n133 = Unbundle By Name(w310) -> ("Sample Settings.USB Port"=w309:refnum<visa-resource-name>)
        n134 = Unbundle By Name(w311) -> ("写/读"=w308:T5, "光功率设置"=w303:u32)
        n135 = call "串口读写 - DS.vi"("寄存器地址"=u8 2, "错误输入（无错误）"=w307, "写入数据"=w303, "写/读"=w308, "VISA输入"=w309) -> ("错误输出"=w306:errorcluster, "读取设备(n)"=w302:i32)  [unwired: 4 in, 1 out]
        n136 = local write "光功率设置"(w302) -> ()
        n137 = call <vilib>:"Add State(s) to Queue__JKI_lib_State_Machine.vi"("State(s) in (\"\")"=w313) -> ("States Out"=w314:string)  [unwired: 14 in]
      }
      frame "---------- API ----------" {
        # "#CSM \"Category Seperator\"\nDo not put any code in this frame."
        n138 = call <vilib>:"Add State(s) to Queue__JKI_lib_State_Machine.vi"("State(s) in (\"\")"=w315) -> ("States Out"=w316:string)  [unwired: 14 in]
      }
      frame "API: Sample Interval" {
        # "#CSM \"Category Seperator\"\nDo not put any code in this frame."
        n139 = call "Convert API String Arguments to Data.vim"("Reference Type"=0.0, "API String"=w321) -> ("Data"=w319:dbl)  [unwired: 6 in, 1 out]
        n140 = call-poly <userlib>:"Build Message with Arguments++.vi"("States With Replace Token"="API: Sample Interval >> <param> ->| Acquisition - <1>" ("State"), "<param>"=w321, "<1>"=w324) -> ("States"=w323:string)  [unwired: 12 in]
        n141 = call <vilib>:"Add State(s) to Queue__JKI_lib_State_Machine.vi"("State(s) in Front (\"\")"=w323, "State(s) in (\"\")"=w326) -> ("States Out"=w327:string)  [unwired: 13 in]
        n142 = Bundle By Name(cluster=w322, "Sample Settings.Interval(s)"=w319) -> (w318:T11)
      }
      frame "API: UDP ONOFF" {
        # "#CSM \"Category Seperator\"\nDo not put any code in this frame."
        n143 = Bundle By Name(cluster=T6 {"连接ID"=refnum, "网络地址(字符串)"="", "地址"=0, "本端口"=12346, "对向"=12345, "Read Interval"=0.15, "Write Interval"=0.15} ("UDP Settings"), "网络地址(字符串)"="地址") -> (w328:T6)
        n144 = call "Convert API String Arguments to Data.vim"("Reference Type"=FALSE, "API String"=w337) -> ("Data"=w331:bool)  [unwired: 6 in, 1 out]
        n145 = local write "UDP"(w331) -> ()
        n146 = call "Convert Data To API String Arguments.vim"("Data"=w328) -> ("API String"=w332:string)  [unwired: 7 in, 1 out]
        n147 = Select(t="API: Start >> <param> ->| UDP - <1>" ("State"), s=w331, f="API: Stop >> <param> ->| UDP - <1>" ("State")) -> (s? t:f=w333:string)
        n148 = call-poly <userlib>:"Build Message with Arguments++.vi"("States With Replace Token"=w333, "<param>"=w332, "<1>"=w340) -> ("States"=w339:string)  [unwired: 12 in]
        n149 = call <vilib>:"Add State(s) to Queue__JKI_lib_State_Machine.vi"("State(s) in Front (\"\")"=w339, "State(s) in (\"\")"=w341) -> ("States Out"=w342:string)  [unwired: 13 in]
      }
      frame "API: UDP Exit" {
        # "#CSM \"Category Seperator\"\nDo not put any code in this frame."
        n150 = local write "UDP"(FALSE ("UDP")) -> ()
        n151 = call-poly <userlib>:"Build Message with Arguments++.vi"("States With Replace Token"="Macro: Exit ->| UDP - <1>" ("State"), "<1>"=w347) -> ("States"=w346:string)  [unwired: 13 in]
        n152 = call <vilib>:"Add State(s) to Queue__JKI_lib_State_Machine.vi"("State(s) in Front (\"\")"=w346, "State(s) in (\"\")"=w348) -> ("States Out"=w349:string)  [unwired: 13 in]
      }
    }
    n153 = Unbundle By Name(w26) -> ("子程序？"=w25:bool)
    n154 = call "State Delete.vi"("Delete?(F)"=w25, "CSM name to delete"=string[] ["Logging"], "State In"=w29) -> ("State Out"=w28:string)  [unwired: 8 in]
  }
  n155 = while {
    shift-right: [w360] -> _
    shift-left: enum16{"Idle", "Initialize", "Exit"}."Initialize" -> [w361]
    tunnel: "CSM Name" -> [w358]
    shift-right: [w356] -> _
    shift-left: w9 -> [w357]
    shift-right: [w354] -> _
    shift-left: -1 -> [w355]
    shift-right: [w353] -> _
    shift-left: _ -> [w352]
    shift-right: [w351] -> _
    shift-left: _ -> [w350]
    stop <- w359 stop-if-true
    n156 = case shown="\"Idle\", 默认" w361 {
      tunnel: [enum16{"Idle", "Initialize", "Exit"}."Idle" w379 enum16{"Idle", "Initialize", "Exit"}."Exit"] -> w360
      tunnel: [_ _ TRUE] -> w359
      tunnel: w358 -> [w365 w378 _]
      tunnel: w357 -> [w368 w376 w462]
      tunnel: [w368 w377 w462] -> w356
      tunnel: w355 -> [_ w374 _]
      tunnel: [-1 w375 _] -> w354
      tunnel: [w364 w372 _] -> w353
      tunnel: w352 -> [_ w373 w461]
      tunnel: [w362 w370 w459] -> w351
      tunnel: w350 -> [_ w371 w459]
      frame "Initialize" {
        w363 = FALSE  # your data
        n157 = call <userlib>:"CSM - Module Exit Event.vi"("Name (\"\" to Use UUID) In"=w365) -> ("CSM Exit Event"=w366:refnum<user-event>)  [unwired: 8 in, 2 out]
        n158 = register-events(w366) -> (reference out=w364:refnum<event-registration>)  [unwired: 2 in, 1 out]
        n159 = Bundle("your data"=w363) -> (w362:cluster{"your data":bool})  [unwired: 1 in]
      }
      frame "Idle", Default {
        n160 = event shown="[5] \"光开关\": 值改变" {
          selector: w373 -> [_ _ _ _ _ _ _ _ _ _]
          dyn-events: [_ _ _ _ _ _ _ _ _ _] -> w372
          timeout: w374 -> [_ _ _ _ _ _ _ _ _ _]
          tunnel: [_ w387 enum16{"Idle", "Initialize", "Exit"}."Exit" _ _ _ _ _ _ _] -> w379
          tunnel: w378 -> [w381 w392 _ _ _ _ _ _ _ _]
          tunnel: w376 -> [w384 _ w401 w407 w416 w424 w433 w442 w447 w456]
          tunnel: [w382 w391 w401 w408 w415 w425 w434 w443 w446 w457] -> w377
          tunnel: [-1 _ _ _ _ _ _ _ _ _] -> w375
          tunnel: w371 -> [w380 w390 w399 w409 w417 w426 w435 w444 w451 w458]
          tunnel: [w380 w390 w399 w409 w417 w426 w435 w444 w451 w458] -> w370
          event Timeout {
            n161 = event-data() -> ()  [unwired: 1 in, 3 out]
            n162 = call-poly <userlib>:"CSM - Filter JKISM String Queue.vi"("States In"=w384) -> ("States Out"=w383:string)  [unwired: 14 in]
            n163 = call <userlib>:"CSM - Forward UI Operations to CSM.vi"("Name (\"\" to Use UUID)"=w381, "State(s) In (\"\")"=w383) -> ("States Out"=w382:string)  [unwired: 8 in, 1 out]
          }
          event Panel Close? {
            n164 = event-data() -> ()  [unwired: 1 in, 1 out]
            n165 = Two Button Dialog(message="确定关闭程序？" ("消息")) -> (T button?=w388:bool)  [unwired: 2 in]
            n166 = case shown="True" w388 {
              tunnel: w392 -> [w394 w397]
              tunnel: [w394 w396] -> w391
              tunnel: [enum16{"Idle", "Initialize", "Exit"}."Idle" enum16{"Idle", "Initialize", "Exit"}."Exit"] -> w387
              frame False {
              }
              frame True {
                n167 = call <userlib>:"CSM - Forward UI Operations to CSM.vi"("Name (\"\" to Use UUID)"=w397, "State(s) In (\"\")"="Macro: Exit" ("State")) -> ("States Out"=w396:string)  [unwired: 8 in, 1 out]
              }
            }
            n168 = event-data("Discard?"=TRUE) -> ()  [unwired: 1 in, 1 out]
          }
          event User Event {
            n169 = event-data() -> ()  [unwired: 1 in, 1 out]
          }
          event "停止": Value Change {
            n170 = event-data() -> ()  [unwired: 1 in, 1 out]
            n171 = Two Button Dialog(message="确定停止程序？" ("消息")) -> (T button?=w404:bool)  [unwired: 2 in]
            n172 = Select(t="Macro: Exit" ("State(s) in Front (\"\")"), s=w404, f="") -> (s? t:f=w402:string)
            n173 = call <vilib>:"Add State(s) to Queue__JKI_lib_State_Machine.vi"("State(s) in Front (\"\")"=w402, "State(s) in (\"\")"=w407) -> ("States Out"=w408:string)  [unwired: 13 in]
          }
          event "距离采集开关": Value Change {
            n174 = event-data() -> ()  [unwired: 1 in, 1 out]
            n175 = Select(t="Macro: Start" ("State(s) in Front (\"\")"), s="距离采集开关", f="Macro: Stop" ("State(s) in Front (\"\")")) -> (s? t:f=w411:string)
            n176 = local write "Error Occurred"(errorcluster {"status"=FALSE, "code"=0, "source"=""} ("错误常量")) -> ()
            n177 = call <vilib>:"Add State(s) to Queue__JKI_lib_State_Machine.vi"("State(s) in Front (\"\")"=w411, "State(s) in (\"\")"=w416) -> ("States Out"=w415:string)  [unwired: 13 in]
          }
          event "光开关": Value Change {
            n178 = event-data() -> ()  [unwired: 1 in, 1 out]
            n179 = Bundle("光开关"="光开关", "写/读"=读写指令类型."06写单个寄存器") -> (w420:cluster{"光开关":bool, "写/读":T5})  [unwired: 1 in]
            n180 = call "Convert Data To API String Arguments.vim"("Data"=w420) -> ("API String"=w423:string)  [unwired: 7 in, 1 out]
            n181 = call <vilib>:"Build State String with Arguments__JKI_lib_State_Machine.vi"("Arguments (\"\")"=w423, "State"="Action: Light ON") -> ("State with Arguments"=w422:string)  [unwired: 4 in]
            n182 = call <vilib>:"Add State(s) to Queue__JKI_lib_State_Machine.vi"("State(s) in Front (\"\")"=w422, "State(s) in (\"\")"=w424) -> ("States Out"=w425:string)  [unwired: 13 in]
          }
          event "光功率模式": Value Change {
            n183 = event-data() -> ()  [unwired: 1 in, 1 out]
            n184 = Bundle("光功率模式"="光功率模式", "写/读"=读写指令类型."06写单个寄存器") -> (w429:cluster{"光功率模式":bool, "写/读":T5})  [unwired: 1 in]
            n185 = call "Convert Data To API String Arguments.vim"("Data"=w429) -> ("API String"=w432:string)  [unwired: 7 in, 1 out]
            n186 = call <vilib>:"Build State String with Arguments__JKI_lib_State_Machine.vi"("Arguments (\"\")"=w432, "State"="Action: Power Mode") -> ("State with Arguments"=w431:string)  [unwired: 4 in]
            n187 = call <vilib>:"Add State(s) to Queue__JKI_lib_State_Machine.vi"("State(s) in Front (\"\")"=w431, "State(s) in (\"\")"=w433) -> ("States Out"=w434:string)  [unwired: 13 in]
          }
          event "光功率设置": Value Change {
            n188 = event-data() -> ()  [unwired: 1 in, 1 out]
            n189 = Bundle("光功率设置"="光功率设置", "写/读"=读写指令类型."06写单个寄存器") -> (w438:cluster{"光功率设置":u32, "写/读":T5})  [unwired: 1 in]
            n190 = call "Convert Data To API String Arguments.vim"("Data"=w438) -> ("API String"=w441:string)  [unwired: 7 in, 1 out]
            n191 = call <vilib>:"Build State String with Arguments__JKI_lib_State_Machine.vi"("Arguments (\"\")"=w441, "State"="Action: Power Num") -> ("State with Arguments"=w440:string)  [unwired: 4 in]
            n192 = call <vilib>:"Add State(s) to Queue__JKI_lib_State_Machine.vi"("State(s) in Front (\"\")"=w440, "State(s) in (\"\")"=w442) -> ("States Out"=w443:string)  [unwired: 13 in]
          }
          event "Interval(s)": Value Change {
            n193 = event-data() -> ()  [unwired: 1 in, 1 out]
            n194 = call "Convert Data To API String Arguments.vim"("Data"="Interval(s)") -> ("API String"=w449:string)  [unwired: 7 in, 1 out]
            n195 = call <vilib>:"Build State String with Arguments__JKI_lib_State_Machine.vi"("Arguments (\"\")"=w449, "State"="API: Sample Interval" ("State(s) in Front (\"\")")) -> ("State with Arguments"=w448:string)  [unwired: 4 in]
            n196 = call <vilib>:"Add State(s) to Queue__JKI_lib_State_Machine.vi"("State(s) in Front (\"\")"=w448, "State(s) in (\"\")"=w447) -> ("States Out"=w446:string)  [unwired: 13 in]
          }
          event "UDP": Value Change {
            n197 = event-data() -> ()  [unwired: 1 in, 1 out]
            n198 = call "Convert Data To API String Arguments.vim"("Data"="UDP") -> ("API String"=w454:string)  [unwired: 7 in, 1 out]
            n199 = call <vilib>:"Build State String with Arguments__JKI_lib_State_Machine.vi"("Arguments (\"\")"=w454, "State"="API: UDP ONOFF" ("State(s) in Front (\"\")")) -> ("State with Arguments"=w453:string)  [unwired: 4 in]
            n200 = call <vilib>:"Add State(s) to Queue__jki_lib_state_machine.vi"("State(s) in Front (\"\")"=w453, "State(s) in (\"\")"=w456) -> ("States Out"=w457:string)  [unwired: 13 in]
          }
        }
      }
      frame "Exit" {
        n201 = Unregister For Events(event registration refnum=w461) -> (error out=w460:errorcluster)  [unwired: 1 in]
        n202 = call <vilib>:"Clear Errors.vi"("error in (no error)"=w460) -> ()  [unwired: 5 in, 2 out]
      }
    }
  }
  n203 = flat-sequence {
    tunnel: w5 -> [_]
    tunnel: "CSM Name" -> [w466]
    tunnel: "子程序？" -> [w468]
    frame #0 {
      n204 = Concatenate Strings("Acquisition - " ("Name(\"\" to use uuid)"), w466) -> (w471:string)
      n205 = call "Acquisition.vi"("CSM Name"=w471) -> ()  [unwired: 11 in]
      n206 = Concatenate Strings("Logging - " ("Name(\"\" to use uuid)"), w466) -> (w469:string)
      n207 = case shown="False" w468 {
        tunnel: w469 -> [w473 _]
        frame False {
          n208 = call "Logging.vi"("CSM Name"=w473) -> ()  [unwired: 11 in]
        }
        frame True {
        }
      }
      n209 = Concatenate Strings("UDP - " ("Name(\"\" to use uuid)"), w466) -> (w465:string)
      n210 = call "CSMclient.vi"("CSM Name"=w465) -> ()  [unwired: 11 in]
    }
  }
  n211 = call <userlib>:"CSM - Sync Configuration Variables to File.vi"("All Temp Variable to Default Ini(F)"=TRUE, "error in (no error)"=w3) -> ()  [unwired: 7 in, 1 out]
